vi "Test - Explain Better Error.vi"() -> ()   [LabVIEW 2020]
uses:
  Explain Error Improved Dialog/Explain Error Improved Dialog.lvlib
panel:
  out "error in (no error)":errorcluster={"status"=FALSE, "code"=7, "source"=""}
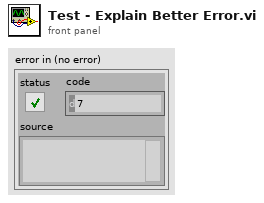
[diagram p1: front panel]
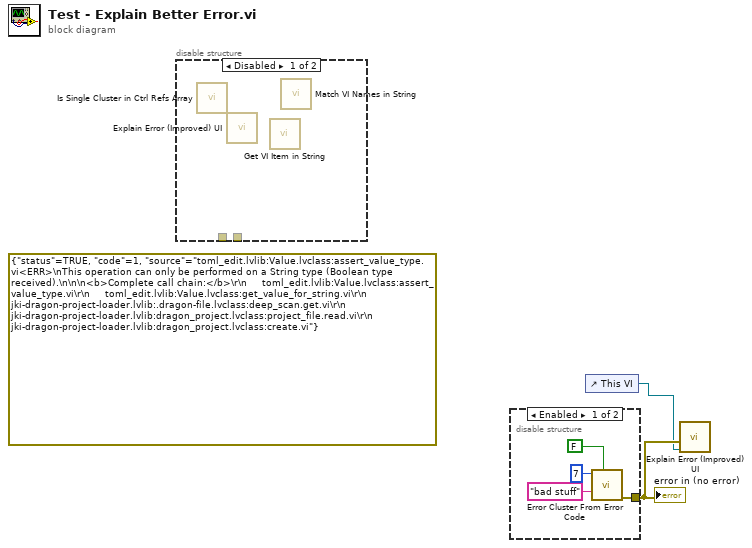
[diagram p0: block diagram]
diagram:
  (unwired) errorcluster {"status"=TRUE, "code"=1, "source"="toml_edit.lvlib:Value.lvclass:assert_value_type.vi<ERR>\nThis operation can only be performed on a String type (Boolean type received).\n\n\n<b>Complete call chain:</b>\r\n     toml_edit.lvlib:Value.lvclass:assert_value_type.vi\r\n     toml_edit.lvlib:Value.lvclass:get_value_for_string.vi\r\n     jki-dragon-project-loader.lvlib:.dragon-file.lvclass:deep_scan.get.vi\r\n     jki-dragon-project-loader.lvlib:dragon_project.lvclass:project_file.read.vi\r\n     jki-dragon-project-loader.lvlib:dragon_project.lvclass:create.vi"} ("Error Cluster")
  n1 = disable-structure shown="Disabled" {
    disable-tunnel: _ -> [w4 _]
    disable-tunnel: _ -> [w3 _]
    frame Disabled {
      n2 = call "Is Single Cluster in Ctrl Refs Array.vi"() -> ()  [unwired: 10 in, 2 out]
      n3 = call "Explain Error (Improved) UI.vi"() -> ()  [unwired: 12 in]
      n4 = call "Get VI Item in String.vi"() -> ()  [unwired: 8 in, 4 out]
      n5 = call "Match VI Names in String.vi"() -> ()  [unwired: 11 in, 1 out]
    }
    frame Enabled {
    }
  }
  n6 = disable-structure shown="Enabled" {
    disable-tunnel: [w8 _] -> w2
    frame Enabled {
      n7 = call <vilib>:"Error Cluster From Error Code.vi"("show call chain? (False)"=FALSE, "error message (\"\")"="bad stuff" ("error message (\"\")"), "error code (0)"=7) -> ("error out"=w8:errorcluster)  [unwired: 6 in]
    }
    frame Disabled {
    }
  }
  "error in (no error)" <- w2
  n8 = control-ref of="This VI"() -> (w1:refnum<vi>)
  n9 = call "Explain Error (Improved) UI.vi"("User VI Ref"=w1, "Error Cluster"=w2) -> ()  [unwired: 10 in]
